vi "GO alerte ecart temperatures.vi"(3 "Numéro":u8) -> (1 "défaut écart températures":bool)   [LabVIEW 2022 SP3]
uses:
  Enum/Enum s1.ctl
  Variables globales/Variable glob alertes ecart temperatures.vi
  Variables globales/Variable glob mails.vi
  Variables globales/Variables glob EUROTHERM.vi
  Variables globales/Variable glob Th.vi
  Variables globales/Variable glob generale.vi
  Variables globales/Variable glob Pt.vi
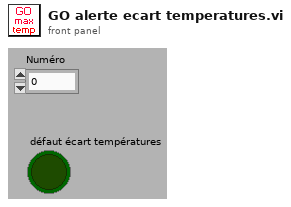
[diagram p1: front panel]
types:
  T1 = typedef "Enum s1.ctl" = enum16{"Alerte vide", "Alerte temperature min-max", "Alerte temperature ecart", "Alerte Keller", "Alerte compteur", "Alerte régulateurs"}
  T2 = cluster{"Indices a controler":i16[], "Defaut":bool, "ecart temp":dbl, "Alerte":bool, ">?":bool, "N°":u16}[]
  T3 = cluster{"Indices a controler":i16[], "Defaut":bool, "ecart temp":dbl, "Alerte":bool, ">?":bool, "N°":u16}
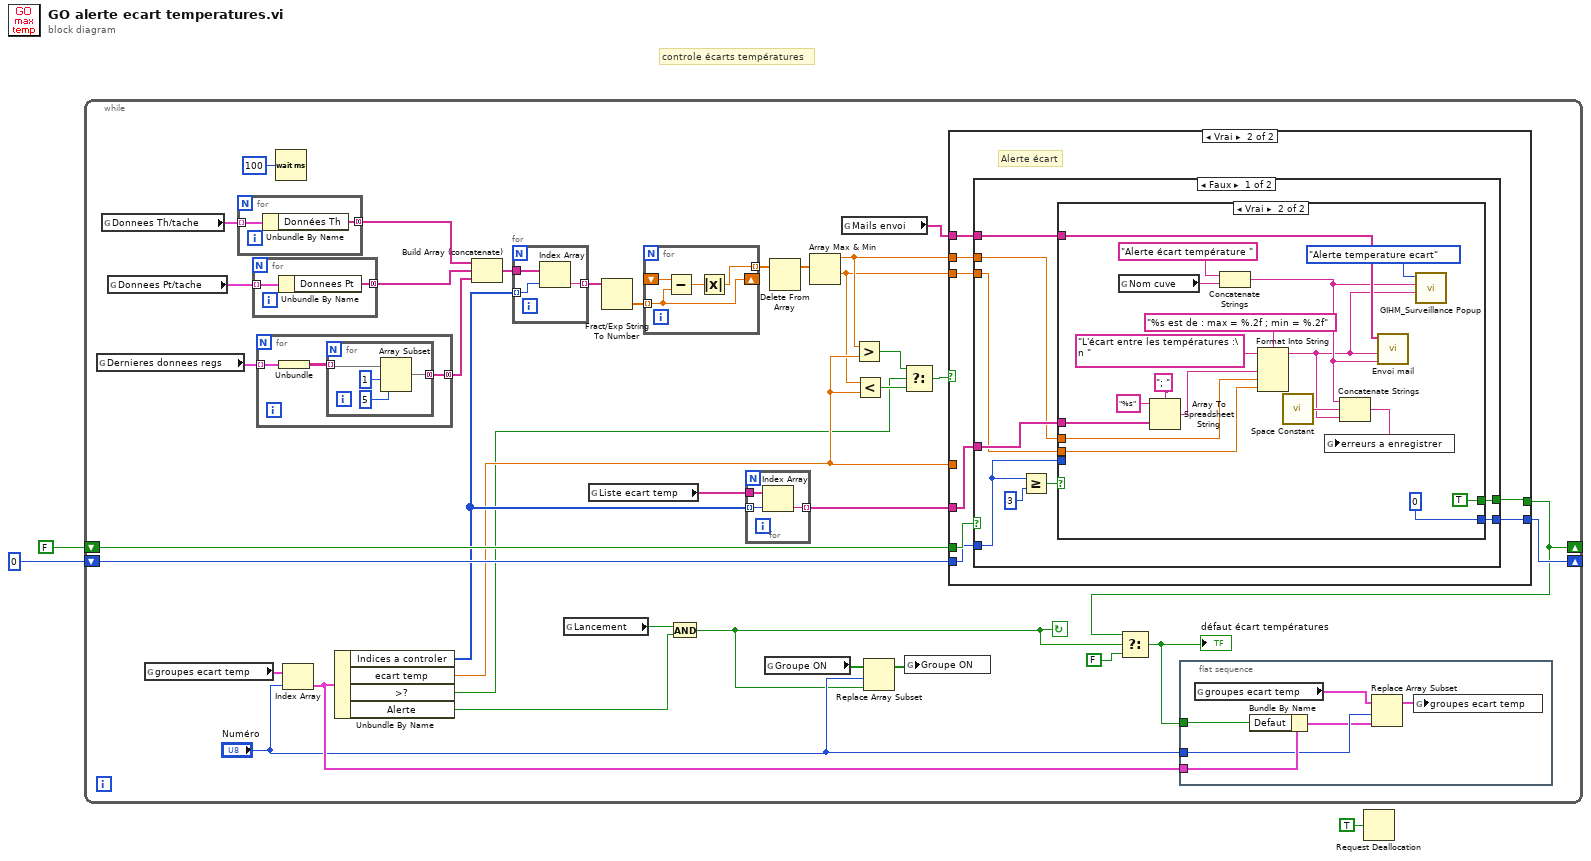
[diagram p0: block diagram]
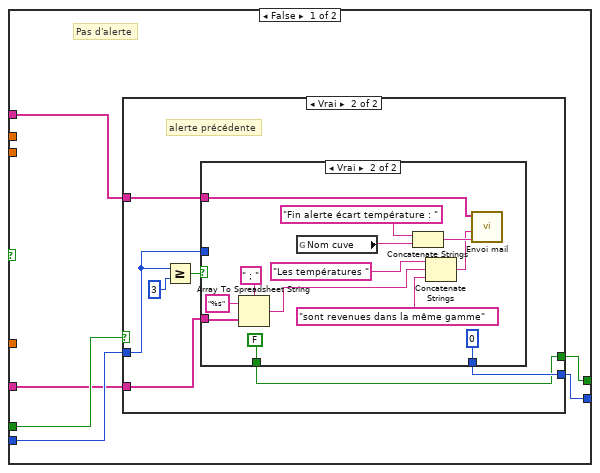
[diagram p2: hidden frame]
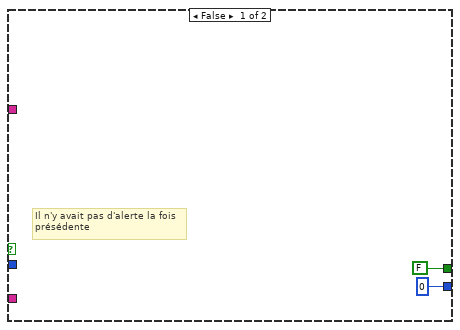
[diagram p3: hidden frame]
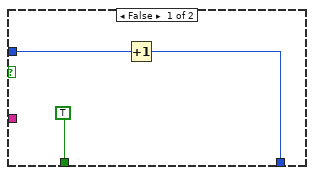
[diagram p4: hidden frame]
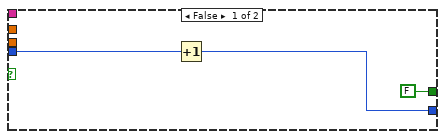
[diagram p5: hidden frame]
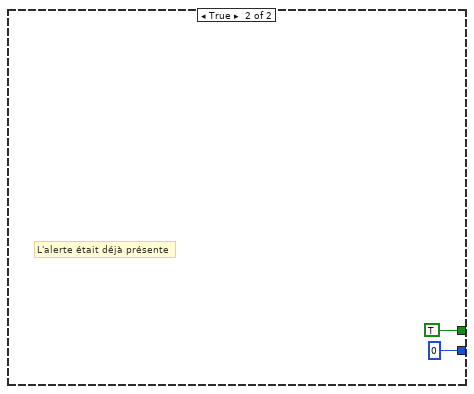
[diagram p6: hidden frame]
diagram:
  # "controle écarts températures"
  n1 = while {
    shift-right: [w25] -> _
    shift-left: FALSE -> [w39]
    shift-right: [w26] -> _
    shift-left: 0 -> [w37]
    stop <- w4 continue-if-true
    n2 = global read "Variables glob EUROTHERM.vi" "Dernieres donnees regs"() -> (w31:cluster{"Dernieres donnees 1COM":string[][]}[])
    n3 = global read "Variable glob Th.vi" "Donnees Th/tache"() -> (w36:cluster{"Données Th":string[]}[])
    n4 = global read "Variable glob Pt.vi" "Donnees Pt/tache"() -> (w34:cluster{"Donnees Pt":string[]}[])
    n5 = global read "Variable glob alertes ecart temperatures.vi" "groupes ecart temp"() -> (w27:T2)
    n6 = for {
      tunnel: w36 -> [w64] mode=indexing
      tunnel: [w63] -> w35 mode=concatenating
      n7 = Unbundle By Name(w64) -> ("Données Th"=w63:string[])
    }
    n8 = for {
      tunnel: w34 -> [w62] mode=indexing
      tunnel: [w61] -> w33 mode=concatenating
      n9 = Unbundle By Name(w62) -> ("Donnees Pt"=w61:string[])
    }
    n10 = for {
      tunnel: w31 -> [w56] mode=indexing
      tunnel: [w54] -> w30 mode=concatenating
      n11 = Unbundle(w56) -> ("Dernieres donnees 1COM"=w55:string[][])
      n12 = for {
        tunnel: w55 -> [w60] mode=indexing
        tunnel: [w57] -> w54 mode=concatenating
        n13 = Array Subset(array=w60, index=1 ("indice"), length=5 ("longueur")) -> (w57:string[])
      }
    }
    n14 = Wait (ms)(milliseconds to wait=u32 100 ("attente (ms)")) -> ()  [unwired: 1 out]
    n15 = Index Array(array=w27, index="Numéro") -> (element=w29:T3)
    n16 = Unbundle By Name(w29) -> ("Indices a controler"=w21:i16[], "ecart temp"=w16:dbl, ">?"=w13:bool, "Alerte"=w9:bool)
    n17 = Build Array (concatenate)(w35, w33, w30) -> (w38:string[])
    n18 = for {
      tunnel: w38 -> [w137]
      tunnel: w21 -> [w138] mode=indexing
      tunnel: [w136] -> w40 mode=indexing
      n19 = Index Array(array=w137, index=w138) -> (element=w136:string)
    }
    n20 = global read "Variable glob generale.vi" "Lancement"() -> (w23:bool)
    n21 = global read "Variable glob alertes ecart temperatures.vi" "Liste ecart temp"() -> (w22:string[])
    n22 = Fract/Exp String To Number(string=w40) -> (number=w19:dbl[])  [unwired: 3 in, 1 out]
    n23 = for {
      tunnel: w19 -> [w42] mode=indexing
      shift-right: [w42] -> _
      shift-left: _ -> [w43]
      tunnel: [w41] -> w18 mode=indexing
      n24 = Subtract(x=w43, y=w42) -> (x-y=w44:dbl)
      n25 = Absolute Value(x=w44) -> (abs(x)=w41:dbl)
    }
    n26 = And(x=w23, y=w9) -> (x .and. y?=w4:bool)
    n27 = for {
      tunnel: w22 -> [w53]
      tunnel: w21 -> [w52] mode=indexing
      tunnel: [w51] -> w20 mode=indexing
      n28 = Index Array(array=w53, index=w52) -> (element=w51:string)
    }
    n29 = global read "Variable glob alertes ecart temperatures.vi" "Groupe ON"() -> (w7:bool[])
    n30 = Delete From Array(array=w18) -> (array with subset deleted=w17:dbl[])  [unwired: 2 in, 1 out]
    n31 = Array Max & Min(array=w17) -> (max value=w11:dbl, min value=w10:dbl)  [unwired: 2 out]
    n32 = global read "Variable glob mails.vi" "Mails envoi"() -> (w8:string[])
    n33 = Greater?(x=w11, y=w16) -> (0:w15:bool)
    n34 = Less?(x=w10, y=w16) -> (x < y?=w14:bool)
    n35 = Replace Array Subset(array=w7, new element=w4, index="Numéro") -> (w5:bool[])
    n36 = Select(t=w15, s=w13, f=w14) -> (s? t:f=w12:bool)
    n37 = global write "Variable glob alertes ecart temperatures.vi" "Groupe ON"(w5) -> ()
    n38 = case shown="Vrai" w12 {
      tunnel: w39 -> [w70 w103]
      tunnel: w8 -> [w69 w102]
      tunnel: w16 -> [_ _]
      tunnel: w37 -> [w68 w101]
      tunnel: [w67 w100] -> w26
      tunnel: [w66 w99] -> w25
      tunnel: w20 -> [w65 w98]
      tunnel: w11 -> [_ w97]
      tunnel: w10 -> [_ w96]
      frame False {
        # "Pas d'alerte"
        n39 = case shown="Vrai" w70 {
          tunnel: w69 -> [_ w79]
          tunnel: w68 -> [_ w78]
          tunnel: [0 w77] -> w67
          tunnel: [FALSE w76] -> w66
          tunnel: w65 -> [_ w73]
          frame False {
            # "Il n'y avait pas d'alerte la fois\nprésédente"
          }
          frame True {
            # "alerte précédente"
            n40 = Greater Or Equal?(x=w78, y=3) -> (x >= y?=w75:bool)
            n41 = case shown="Vrai" w75 {
              tunnel: w79 -> [_ w94]
              tunnel: [TRUE FALSE] -> w76
              tunnel: [w81 0] -> w77
              tunnel: w78 -> [w82 _]
              tunnel: w73 -> [_ w89]
              frame False {
                n42 = Increment(x=w82) -> (x+1=w81:i32)
              }
              frame True {
                n43 = Array To Spreadsheet String(delimiter (Tab)=" ; " ("séparateur (Tabulation)"), array=w89, 3:"%s" ("chaîne de format")) -> (spreadsheet string=w85:string)
                n44 = global read "Variable glob generale.vi" "Nom cuve"() -> (w90:string)
                n45 = Concatenate Strings("Fin alerte écart température : " ("subject ([No Subject])"), w90) -> (w93:string)
                n46 = Concatenate Strings("Les températures ", w85, "sont revenues dans la même gamme") -> (w83:string)
                n47 = call "Envoi mail.vi"("Objet"=w93, "Message"=w83, "Mail liste"=w94) -> ()  [unwired: 3 in]
              }
            }
          }
        }
      }
      frame True {
        # "Alerte écart"
        n48 = case shown="Faux" w103 {
          tunnel: w102 -> [w112 _]
          tunnel: w101 -> [w109 _]
          tunnel: [w108 0] -> w100
          tunnel: [w107 TRUE] -> w99
          tunnel: w98 -> [w106 _]
          tunnel: w97 -> [w105 _]
          tunnel: w96 -> [w104 _]
          frame False {
            n49 = Greater Or Equal?(x=w109, y=3) -> (x >= y?=w110:bool)
            n50 = case shown="Vrai" w110 {
              tunnel: w112 -> [_ w132]
              tunnel: w109 -> [w115 _]
              tunnel: [w114 0] -> w108
              tunnel: [FALSE TRUE] -> w107
              tunnel: w106 -> [_ w125]
              tunnel: w105 -> [_ w122]
              tunnel: w104 -> [_ w121]
              frame False {
                n51 = Increment(x=w115) -> (x+1=w114:i32)
              }
              frame True {
                n52 = global read "Variable glob generale.vi" "Nom cuve"() -> (w128:string)
                n53 = Array To Spreadsheet String(delimiter (Tab)="; " ("séparateur (Tabulation)"), array=w125, 3:"%s" ("chaîne de format")) -> (spreadsheet string=w123:string)
                n54 = Concatenate Strings("Alerte écart température " ("subject ([No Subject])"), w128) -> (w118:string)
                n55 = Format Into String(format string="%s est de : max = %.2f ; min = %.2f" ("chaîne de format"), initial string="L'écart entre les températures :\n ", w123, w122, w121) -> (resulting string=w117:string)  [unwired: 1 in, 1 out]
                n56 = call <vilib>:"Space Constant.vi"() -> ("String"=w119:string)
                n57 = Concatenate Strings(w118, w119, w117) -> (w131:string)
                n58 = global write "Variable glob generale.vi" "erreurs a enregistrer"(w131) -> ()
                n59 = call "Envoi mail.vi"("Objet"=w118, "Message"=w117, "Mail liste"=w132) -> ()  [unwired: 3 in]
                n60 = call "GIHM_Surveillance Popup.vi"("Message"=w117, "Problème observé"=w118, "Type problème"=Enum_s1."Alerte temperature ecart") -> ()  [unwired: 2 in, 1 out]
              }
            }
          }
          frame True {
            # "L'alerte était déjà présente"
          }
        }
      }
    }
    n61 = Select(t=w25, s=w4, f=FALSE ("cas faux")) -> (s? t:f=w28:bool)
    "défaut écart températures" <- w28
    n62 = flat-sequence {
      tunnel: w29 -> [w50]
      tunnel: w28 -> [w49]
      tunnel: "Numéro" -> [w48]
      frame #0 {
        n63 = global read "Variable glob alertes ecart temperatures.vi" "groupes ecart temp"() -> (w45:T2)
        n64 = Bundle By Name(cluster=w50, "Defaut"=w49) -> (w47:T3)
        n65 = Replace Array Subset(array=w45, new element=w47, index=w48) -> (w46:T2)
        n66 = global write "Variable glob alertes ecart temperatures.vi" "groupes ecart temp"(w46) -> ()
      }
    }
  }
  n67 = Request Deallocation(TRUE ("flag")) -> ()
